vi "Month File Name.vi"(8 "error in (no error)":errorcluster, 11 "Start Time":timestamp) -> (0 "error out":errorcluster, 3 "File Name":string)   [LabVIEW 2024]
doc: "Returns the name of the month file a time entry belongs in - YYYY-MM.ini - taken from its Start Time IN UTC. It never looks at the current date: an entry that starts on 30 September 23:30 UTC goes into 2025-09.ini even when it is saved in October.\n\nGenerated by: Claude"
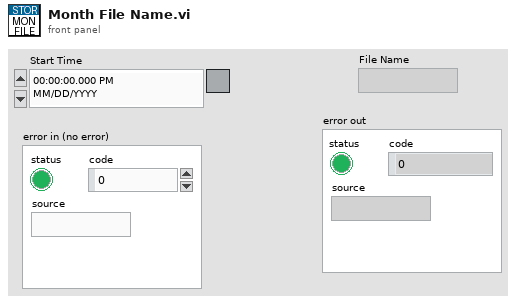
[diagram p1: front panel]
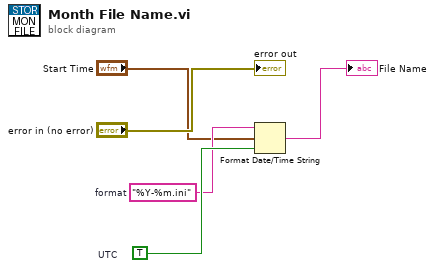
[diagram p0: block diagram]
diagram:
  w4 = TRUE  # UTC
  w3 = "%Y-%m.ini"  # format
  n1 = Format Date/Time String(time format string (%c)=w3, seconds (now)="Start Time", UTC format=w4) -> (date/time string=→"File Name":string)
  "error out" <- "error in (no error)"
